vi "Generate Mock Class.vi"(6 "Add to lvproj?":bool=TRUE, 8 "error in (no error)":errorcluster, 9 "Destination Class Path":path=path "C:/Users/AntonSundqvist/Desktop/temp/test.lvclass", 10 "Source Class Path":path=path "C:/git/astemes-lmock/tests/Test Doubles/Test Interface/Test Interface.lvclass") -> (0 "error out":errorcluster, 2 "Created Files":path[](array[path]))   [LabVIEW 2020, in "Mock Class Generator.lvclass"]
uses:
  Mock Class Generator.lvclass
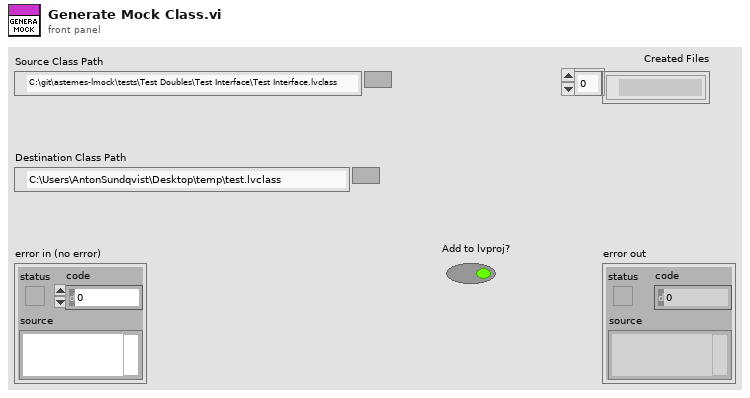
[diagram p1: front panel]
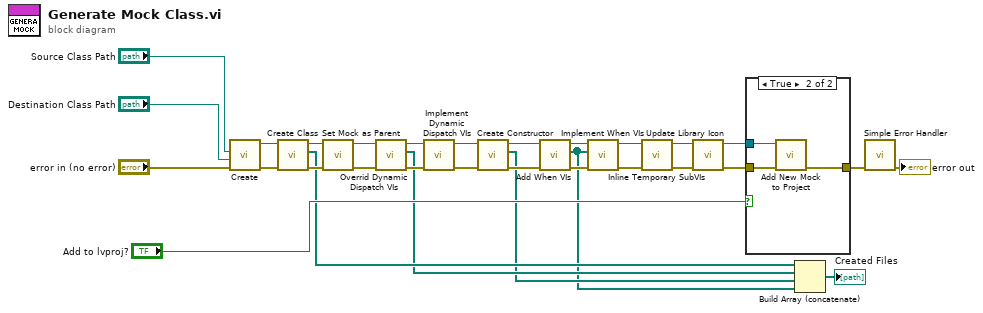
[diagram p0: block diagram]
diagram:
  n1 = call "Create.vi"("error in (no error)"="error in (no error)", "Destination Class Path"="Destination Class Path", "Source Class Path"="Source Class Path") -> ("error out"=w29:errorcluster, "Mock Class Generator Out"=w30:refnum<class "Mock Class Generator.lvclass">)  [unwired: 7 in]
  n2 = call "Create Class.vi"("error in (no error)"=w29, "Mock Class Generator in"=w30) -> ("error out"=w19:errorcluster, "Created Class"=w5:path[], "Mock Class Generator out"=w21:refnum<class "Mock Class Generator.lvclass">)  [unwired: 7 in]
  n3 = call "Set Mock as Parent.vi"("error in (no error)"=w19, "Mock Class Generator in"=w21) -> ("error out"=w18:errorcluster, "Mock Class Generator out"=w20:refnum<class "Mock Class Generator.lvclass">)  [unwired: 8 in]
  n4 = call "Overrid Dynamic Dispatch VIs.vi"("error in (no error)"=w18, "Mock Class Generator in"=w20) -> ("error out"=w25:errorcluster, "Created VI:s"=w4:path[], "Mock Class Generator out"=w26:refnum<class "Mock Class Generator.lvclass">)  [unwired: 7 in]
  n5 = call "Implement Dynamic Dispatch VIs.vi"("error in (no error)"=w25, "Mock Class Generator In"=w26) -> ("error out"=w24:errorcluster, "Mock Class Generator Out"=w22:refnum<class "Mock Class Generator.lvclass">)  [unwired: 8 in]
  n6 = call "Create Constructor.vi"("error in (no error)"=w24, "Mock Class Generator in"=w22) -> ("error out"=w16:errorcluster, "Created Constructor"=w3:path[], "Mock Class Generator"=w15:refnum<class "Mock Class Generator.lvclass">)  [unwired: 7 in]
  n7 = call "Add When VIs.vi"("error in (no error)"=w16, "Mock Class Generator In"=w15) -> ("error out"=w14:errorcluster, "When VIs"=w2:path[], "Mock Class Generator Out"=w12:refnum<class "Mock Class Generator.lvclass">)  [unwired: 7 in]
  n8 = call "Implement When VIs.vi"("error in (no error)"=w14, "When VIs"=w2, "Mock Class Generator In"=w12) -> ("error out"=w13:errorcluster, "Mock Class Generator Out"=w10:refnum<class "Mock Class Generator.lvclass">)  [unwired: 7 in]
  n9 = call "Inline Temporary SubVIs.vi"("error in (no error)"=w13, "Responsive Mock Class Generator in"=w10) -> ("error out"=w8:errorcluster, "Responsive Mock Class Generator out"=w7:refnum<class "Mock Class Generator.lvclass">)  [unwired: 8 in]
  n10 = call "Update Library Icon.vi"("error in (no error)"=w8, "Mock Class Generator In"=w7) -> ("error out"=w11:errorcluster, "Mock Class Generator Out"=w9:refnum<class "Mock Class Generator.lvclass">)  [unwired: 8 in]
  n11 = case shown="True" "Add to lvproj?" {
    tunnel: w11 -> [w32 w35]
    tunnel: [w32 w34] -> w23
    tunnel: w9 -> [_ w33]
    frame False {
    }
    frame True {
      n12 = call "Add New Mock to Project.vi"("error in (no error)"=w35, "Mock Class Generator in"=w33) -> ("error out"=w34:errorcluster)  [unwired: 8 in, 1 out]
    }
  }
  n13 = Build Array (concatenate)(w5, w4, w3, w2) -> (→"Created Files":path[])
  n14 = call <vilib>:"Simple Error Handler.vi"("error in (no error)"=w23) -> ("error out"=→"error out":errorcluster)  [unwired: 4 in, 4 out]
